vi "Write to Hardware.vi"(7 "valid triggers":bool, 8 "error in":errorcluster, 9 "trigger values":dbl[](array[numeric]), 10 "Values in":dbl[](array[numeric]), 11 "Ballard ARINC-429 Tx Execution Unit in":refnum<class "Tx Scheduled Labels Execution Unit.lvclass">) -> (0 "error out":errorcluster, 1 "trigger values out":dbl[](array[numeric]), 2 "Values out":dbl[](array[numeric]), 3 "Ballard ARINC-429 Tx Execution Unit out":refnum<class "Tx Scheduled Labels Execution Unit.lvclass">)   [LabVIEW 2020, in "Ballard ARINC 429 Engine.lvlib" / "Implementation.lvlib" / "Tx Scheduled Labels Execution Unit.lvclass"]
uses:
  Tx Scheduled Labels Execution Unit.lvclass
  Tx Scheduled Labels Execution Unit.lvclass/Tx Scheduled Labels Execution Unit.ctl
  Custom Device/Write Error to System Log.vi/ca55ed61-c1f5-4d13-8aef-490b87d2cf89.vi
  Shared/Encode Parameter and Update Word (32-bit).vi/1445f95d-237d-4fc6-96b9-8992d347f513.vi
  Shared/Encode Parameter and Update Word (32-bit).vi/6b8853f0-8e5d-49e3-9391-4d3f8e5314b0.vi
  Shared/Encode Parameter and Update Word (32-bit).vi/2babc4f4-546e-4d35-846d-a4a1fbac0249.vi
  Shared/Encode Parameter and Update Word (32-bit).vi/1445f95d-237d-4fc6-96b9-8992d347f513.vi/9377bb8f-44b5-4a8f-87f1-966fd5a9edcc.vi
  Shared/Encode Parameter and Update Word (32-bit).vi/1445f95d-237d-4fc6-96b9-8992d347f513.vi/e95d9d1f-307c-44d6-9f26-c3f519a4990d.vi
  Shared/Encode Parameter and Update Word (32-bit).vi/1445f95d-237d-4fc6-96b9-8992d347f513.vi/0c23f515-4369-4514-bc3d-4444e6b437b2.vi
  Shared/Encode Parameter and Update Word (32-bit).vi/6b8853f0-8e5d-49e3-9391-4d3f8e5314b0.vi/136dcdcb-2dd3-4a4d-a796-a8f7a3f8e1ac.vi
  Shared/Encode Parameter and Update Word (32-bit).vi/6b8853f0-8e5d-49e3-9391-4d3f8e5314b0.vi/a54b505c-1216-4ef4-8378-3ceda9d188df.vi
  <vilib>/NI/NI VeriStand Encoding and Decoding/Get Bits Per Digit from Base.vi
  <vilib>/NI VeriStand/Custom Device Tools/Custom Device Utility Library/NI VeriStand - Print Debug Line.vi
  Custom Device/Custom Device.lvlib
  Hardware API/Ballard ARINC 429 Hardware API.lvlib
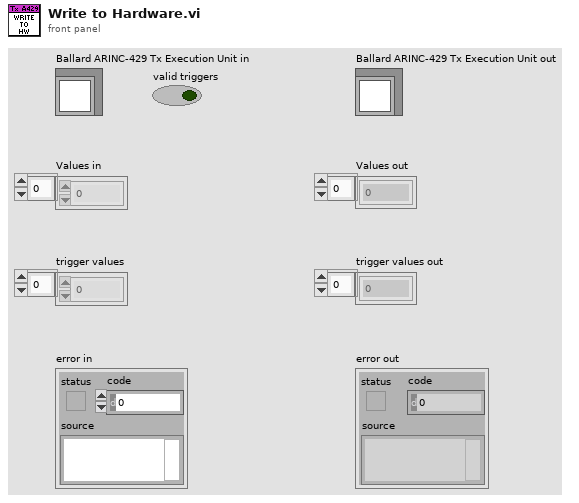
[diagram p1: front panel]
types:
  T1 = typedef "RT Hardware Channel Settings.ctl" = cluster{"channel #":u16, "channel handle":u64, "labels settings for RT":T2[]}
  T2 = typedef "RT Label Settings.ctl" = cluster{"Name":string, "xmlName":string, "label":T3, "transfer period":u32, "SDI_Enabled":bool, "SDI":u8, "parameter driver data":T4, "transfer type":T8, "has timestamp?":bool, "Label Disable/Trigger Channel Reference":T7, "Message Handle":u64, "Initialized?":bool, "Word Initial Raw Value":u32, "Label Timestamp Channel Data Reference":T9, "disabled":bool}
  T3 = typedef "Label.ctl" = u8
  T4 = typedef "RT Parameters.ctl" = cluster{"parameter definitions":T5[], "Tx parameter refs":T7[]}
  T5 = typedef "Parameter Definition.ctl" = cluster{"start index":i32, "size":i32, "encoding":T6, "signed":bool, "scale multiplier":dbl, "scale offset":dbl}
  T6 = typedef "Encoding and Decoding.lvlib/Encoding.ctl" = enum16{"BNR", "BCD", "Discrete"}
  T7 = typedef "Custom Device API.lvlib/Custom Device Item Ref.ctl" = u64
  T8 = typedef "Transfer Type.ctl" = enum16{"Scheduled", "Acyclic", "Block", "Strobe"}
  T9 = typedef "Custom Device API.lvlib/Data Reference.ctl" = i32
  T10 = typedef "Map of Values Indexes to Channel and Label Indexes.ctl" = map{i32, cluster{"channel index":i32, "label index":i32, "group values start index":i32, "values in group":i32}}
  T11 = cluster{"channel index":i32, "label index":i32, "group values start index":i32, "values in group":i32}
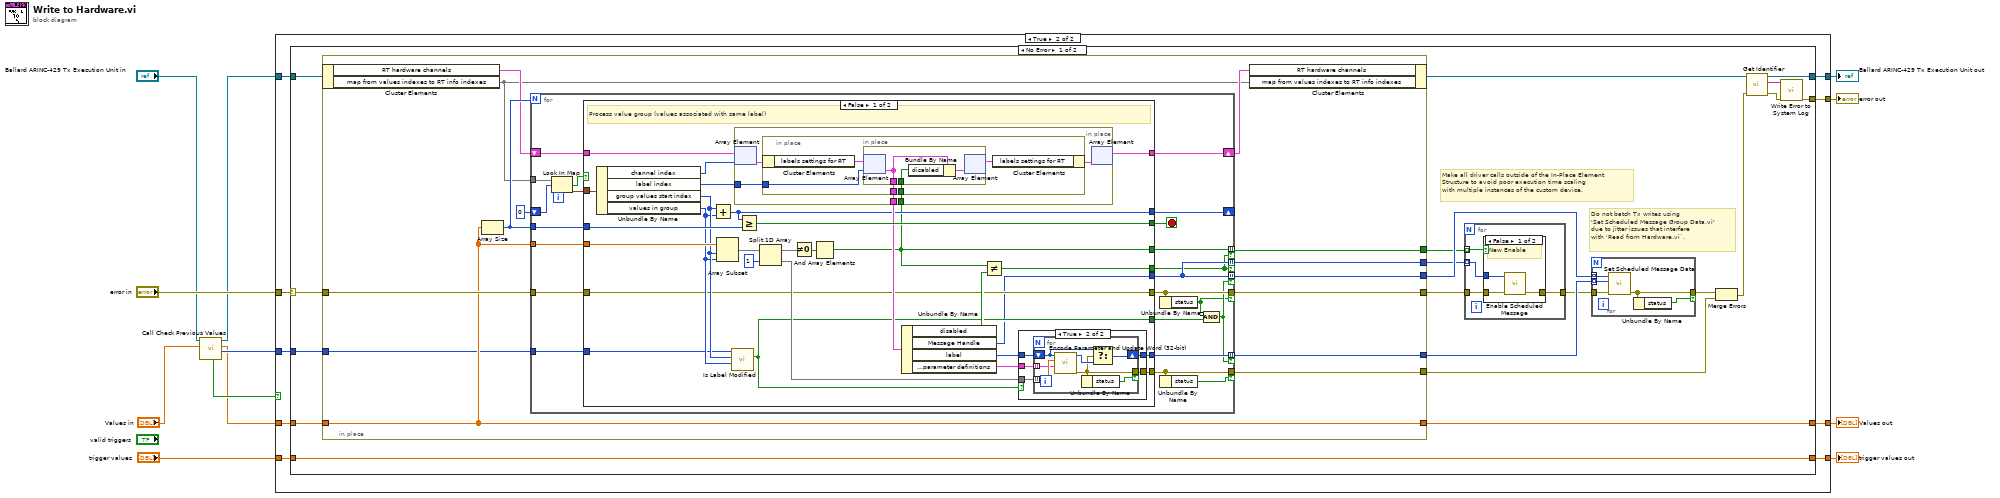
[diagram p0: block diagram]
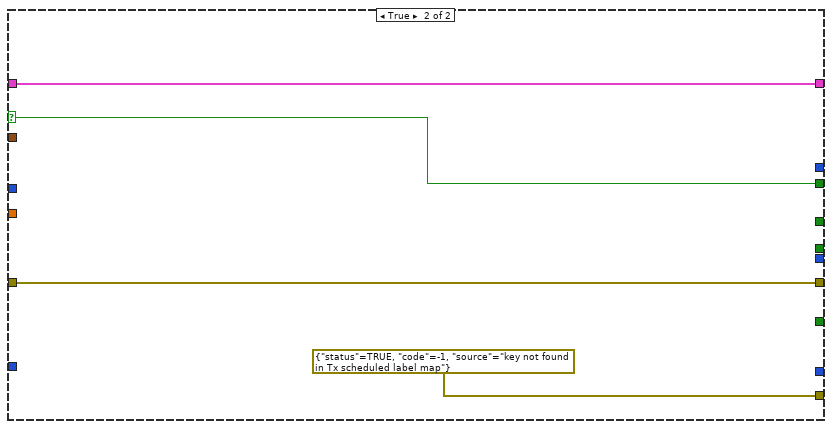
[diagram p4: hidden frame]
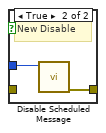
[diagram p5: hidden frame]
diagram:
  n1 = call "Call Check Previous Values.vi"("values"="Values in", "Tx Scheduled Labels Execution Unit in"="Ballard ARINC-429 Tx Execution Unit in") -> ("modified indices"=w4:i32[], "values out"=w1:dbl[], "Tx Scheduled Labels Execution Unit out"=w2:refnum<class "Tx Scheduled Labels Execution Unit.lvclass">, "values modified?"=w5:bool)  [unwired: 5 in, 1 out]
  n2 = case shown="True" w5 {
    tunnel: [w14 w25] -> w12
    tunnel: "error in" -> [w14 w24]
    tunnel: [w15 w23] -> w10
    tunnel: [w13 w22] -> w9
    tunnel: w2 -> [w13 w21]
    tunnel: [w16 w20] -> w8
    tunnel: "trigger values" -> [w16 w19]
    tunnel: w1 -> [w15 w18]
    tunnel: w4 -> [_ w17]
    frame False {
      # "If the Values in have not changed since the last call to Write to Hardware, skip the Write to Hardware step"
    }
    frame True {
      n3 = case shown="No Error" w24 {
        selector: w24 -> [w38 w156]
        tunnel: [w39 w156] -> w25
        tunnel: [w32 w155] -> w23
        tunnel: w18 -> [w45 w155]
        tunnel: [w40 w157] -> w22
        tunnel: w21 -> [w33 w157]
        tunnel: [w42 w154] -> w20
        tunnel: w19 -> [w42 w154]
        tunnel: w17 -> [w31 _]
        frame No Error {
          # "Make all driver calls outside of the In-Place Element\nStructure to avoid poor execution time scaling\nwith multiple instances of the custom device."
          # "Do not batch Tx writes using\n'Set Scheduled Message Group Data.vi'\ndue to jitter issues that interfere\nwith 'Read from Hardware.vi`."
          n4 = in-place {
            in-place-border: [w59] -> w28
            in-place-border: w45 -> [w49]
            in-place-border: [w56] -> w30
            in-place-border: [w55] -> w44
            in-place-border: [w54] -> w43
            in-place-border: w38 -> [w53]
            in-place-border: [w49] -> w32
            in-place-border: w31 -> [w48]
            in-place-border: [w47] -> w27
            in-place-border: [w46] -> w26
            n5 = in-place-cluster #1(w33) -> ("RT hardware channels"=w52:T1[], "map from values indexes to RT info indexes"=w50:T10)
            n6 = Array Size(array=w49) -> (size(s)=w57:i32)
            n7 = for {
              N: w57 -> [_]
              tunnel: w49 -> [w76]
              tunnel: [w81] -> w54 mode=indexing if=w65
              tunnel: [w62] -> w59 mode=indexing if=w65
              tunnel: w50 -> [w79]
              shift-right: [w74] -> _
              shift-left: 0 -> [w78]
              tunnel: w57 -> [w75]
              shift-right: [w71] -> w51
              shift-left: w52 -> [w80]
              tunnel: w53 -> [w70]
              tunnel: [w67] -> w56 if=w63
              tunnel: [w69] -> w55 if=w68
              tunnel: w48 -> [w66]
              tunnel: [w62] -> w46 mode=indexing if=w60
              tunnel: [w61] -> w47 mode=indexing if=w60
              stop <- w72 stop-if-true
              n8 = Look In Map(map=w79, key=w78) -> (key not found?=w73:bool, value=w77:T11)  [unwired: 1 in]
              n9 = case shown="False" w73 {
                selector: w73 -> [_ w139]
                tunnel: [w105 _] -> w81
                tunnel: w70 -> [w86 w137]
                tunnel: [w90 errorcluster {"status"=TRUE, "code"=-1, "source"="key not found in Tx scheduled label map"} ("error in")] -> w69
                tunnel: [w85 _] -> w62
                tunnel: w80 -> [w94 w138]
                tunnel: w77 -> [w109 _]
                tunnel: w76 -> [w108 _]
                tunnel: w75 -> [w107 _]
                tunnel: [w95 _] -> w74
                tunnel: [w106 w139] -> w72
                tunnel: [w92 w138] -> w71
                tunnel: [w86 w137] -> w67
                tunnel: w66 -> [w82 _]
                tunnel: [w87 _] -> w64
                tunnel: [w84 _] -> w60
                tunnel: [w83 _] -> w61
                frame False {
                  # "Process value group (values associated with same label)"
                  n10 = Unbundle By Name(w109) -> ("channel index"=w93:i32, "label index"=w96:i32, "group values start index"=w89:i32, "values in group"=w88:i32)
                  n11 = Add(x=w89, y=w88) -> (x+y=w95:i32)
                  n12 = Array Subset(array=w108, index=w89, length=w88) -> (w103:dbl[])
                  n13 = call "Is Label Modified.vi"("number of parameters"=w88, "initial index"=w89, "modified indices"=w82) -> ("label modified"=w87:bool)  [unwired: 8 in]
                  n14 = Greater Or Equal?(x=w95, y=w107) -> (x >= y?=w106:bool)
                  n15 = Split 1D Array(array=w103, index=1) -> (first subarray=w102:dbl[], second subarray=w91:dbl[])
                  n16 = Not Equal To 0?(x=w102) -> (x != 0?=w101:bool[])
                  n17 = And Array Elements(Boolean array=w101) -> (logical AND=w83:bool)
                  n18 = in-place {
                    in-place-border: [w127] -> w97
                    in-place-border: w83 -> [w126]
                    in-place-border: w96 -> [w125]
                    n19 = in-place-array #2(w94, w93) -> (w123:T1)
                    n20 = in-place {
                      in-place-border: [w132] -> w127
                      in-place-border: w126 -> [w131]
                      in-place-border: w125 -> [w130]
                      n21 = in-place-cluster #3(w123) -> ("labels settings for RT"=w129:T2[])
                      n22 = in-place {
                        in-place-border: [w134] -> w132
                        in-place-border: w131 -> [w135]
                        n23 = in-place-array #4(w129, w130) -> (w134:T2)
                        n24 = Bundle By Name(cluster=w134, "disabled"=w135) -> (w133:T2)
                        n25 = in-place-array #4(w133) -> (w128:T2[])  [unwired: 1 out]
                      }
                      n26 = in-place-cluster #3("labels settings for RT"=w128) -> (w124:T1)
                    }
                    n27 = in-place-array #2(w124) -> (w92:T1[])  [unwired: 1 out]
                  }
                  n28 = Unbundle By Name(w97) -> ("disabled"=w98:bool, "Message Handle"=w85:u64, "label"=w99:T3, "parameter driver data.parameter definitions"=w100:T5[])
                  n29 = Not Equal?(x=w83, y=w98) -> (x != y?=w84:bool)
                  n30 = case shown="True" w87 {
                    tunnel: [w110 w115] -> w105
                    tunnel: w100 -> [_ w114]
                    tunnel: w99 -> [w110 w113]
                    tunnel: w91 -> [_ w112]
                    tunnel: [_ w111] -> w90
                    frame False {
                    }
                    frame True {
                      n31 = for {
                        tunnel: w112 -> [w122] mode=indexing
                        shift-right: [w119] -> w115
                        shift-left: w113 -> [w120]
                        tunnel: w114 -> [w121] mode=indexing
                        tunnel: [w117] -> w111 if=w116
                        n32 = call "Encode Parameter and Update Word (32-bit).vi"("parameter definition"=w121, "parameter value"=w122, "word in"=w120) -> ("error out"=w117:errorcluster, "word out"=w118:u32)  [unwired: 7 in]
                        n33 = Unbundle By Name(w117) -> ("status"=w116:bool)
                        n34 = Select(t=w120, s=w117, f=w118) -> (s? t:f=w119:u32)
                      }
                    }
                  }
                }
                frame True {
                }
              }
              n35 = Unbundle By Name(w67) -> ("status"=w63:bool)
              n36 = Unbundle By Name(w69) -> ("status"=w68:bool)
              n37 = Compound Arithmetic op=AND(invert w63, w64) -> (w65:bool)
            }
            n38 = in-place-cluster #1("RT hardware channels"=w51, "map from values indexes to RT info indexes"=w50) -> (w36:refnum<class "Tx Scheduled Labels Execution Unit.lvclass">)
          }
          n39 = for {
            tunnel: w30 -> [w143]
            tunnel: [w142] -> w29
            tunnel: w27 -> [w141] mode=indexing
            tunnel: w26 -> [w140] mode=indexing
            n40 = case shown="False" w141 {
              tunnel: w140 -> [w146 w148]
              tunnel: [w145 w147] -> w142
              tunnel: w143 -> [w144 _]
              frame False {
                # "New Enable"
                n41 = call "Enable Scheduled Message.vi"("error in (no error)"=w144, "message handle in"=w146) -> ("error out"=w145:errorcluster)  [unwired: 8 in, 1 out]
              }
              frame True {
                # "New Disable"
                n42 = call "Disable Scheduled Message.vi"("message handle in"=w148) -> ("error out"=w147:errorcluster)  [unwired: 9 in, 1 out]
              }
            }
          }
          n43 = for {
            tunnel: w28 -> [w151] mode=indexing
            tunnel: w43 -> [w153] mode=indexing
            tunnel: w29 -> [w152]
            tunnel: [w150] -> w37 if=w149
            n44 = call "Set Scheduled Message Data.vi"("error in (no error)"=w152, "value"=w153, "message handle in"=w151) -> ("error out"=w150:errorcluster)  [unwired: 7 in, 1 out]
            n45 = Unbundle By Name(w150) -> ("status"=w149:bool)
          }
          n46 = Merge Errors(w37, w44) -> (w35:errorcluster)
          n47 = call-dynamic "Get Identifier.vi"("error in"=w35, "Ballard ARINC-429 Execution Unit in"=w36) -> ("error out"=w34:errorcluster, "identifier"=w41:string, "Ballard ARINC-429 Execution Unit out"=w40:refnum<class "Tx Scheduled Labels Execution Unit.lvclass">)  [unwired: 7 in]
          n48 = call "Write Error to System Log.vi"("error in"=w34, "identifier"=w41) -> ("error out"=w39:errorcluster)  [unwired: 9 in]
        }
        frame Error {
        }
      }
    }
  }
  "error out" <- w12
  "Ballard ARINC-429 Tx Execution Unit out" <- w9
  "Values out" <- w10
  "trigger values out" <- w8
